vi "485AAA.vi"() -> ()   [LabVIEW 2024]
uses:
  <vilib>/Utility/file.llb/Write Delimited Spreadsheet (string).vi
  <vilib>/Instr/_visa.llb/VISA Configure Serial Port (Instr).vi
panel:
  out "错误输出":errorcluster
  in  "停止":bool
  out "读取缓冲区":string
  out "返回数":u32
  out "波形图表":dbl(graph)
  out "瞬时流量":dbl
  in  "stop bits (10: 1 bit)":u16(ring)=10 caption="停止位（10: 1位）" items=["1.0"=10, "1.5"=15, "2.0"=20]
  in  "parity (0:none)":enum16{"None", "Odd", "Even", "Mark", "Space"}(ring) caption="奇偶（0:无）"
  in  "baud rate (9600)":u32=9600 caption="波特率(9600)"
  in  "VISA resource name":refnum<visa-resource-name> caption="VISA资源名称"
  out "dup path":path caption="路径副本"
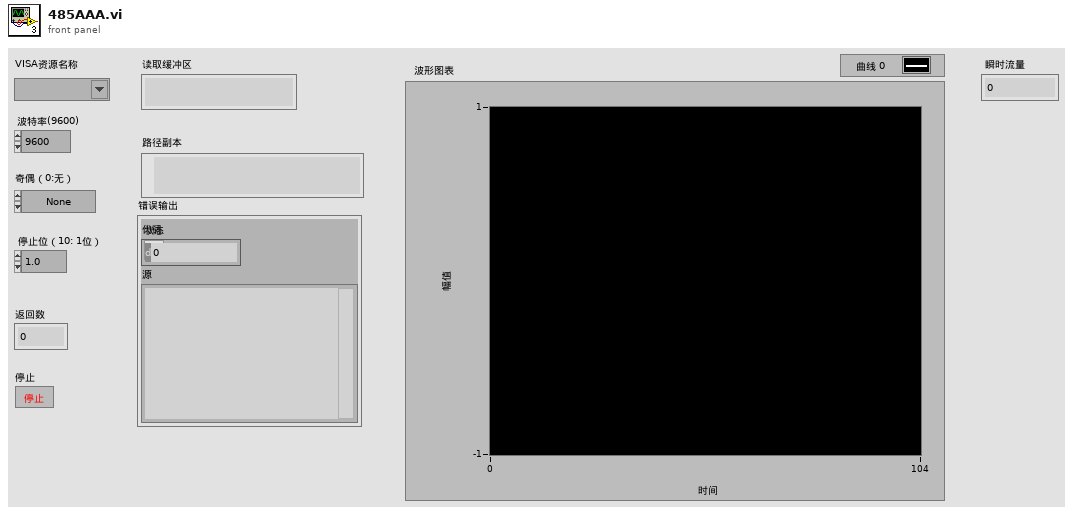
[diagram p1: front panel]
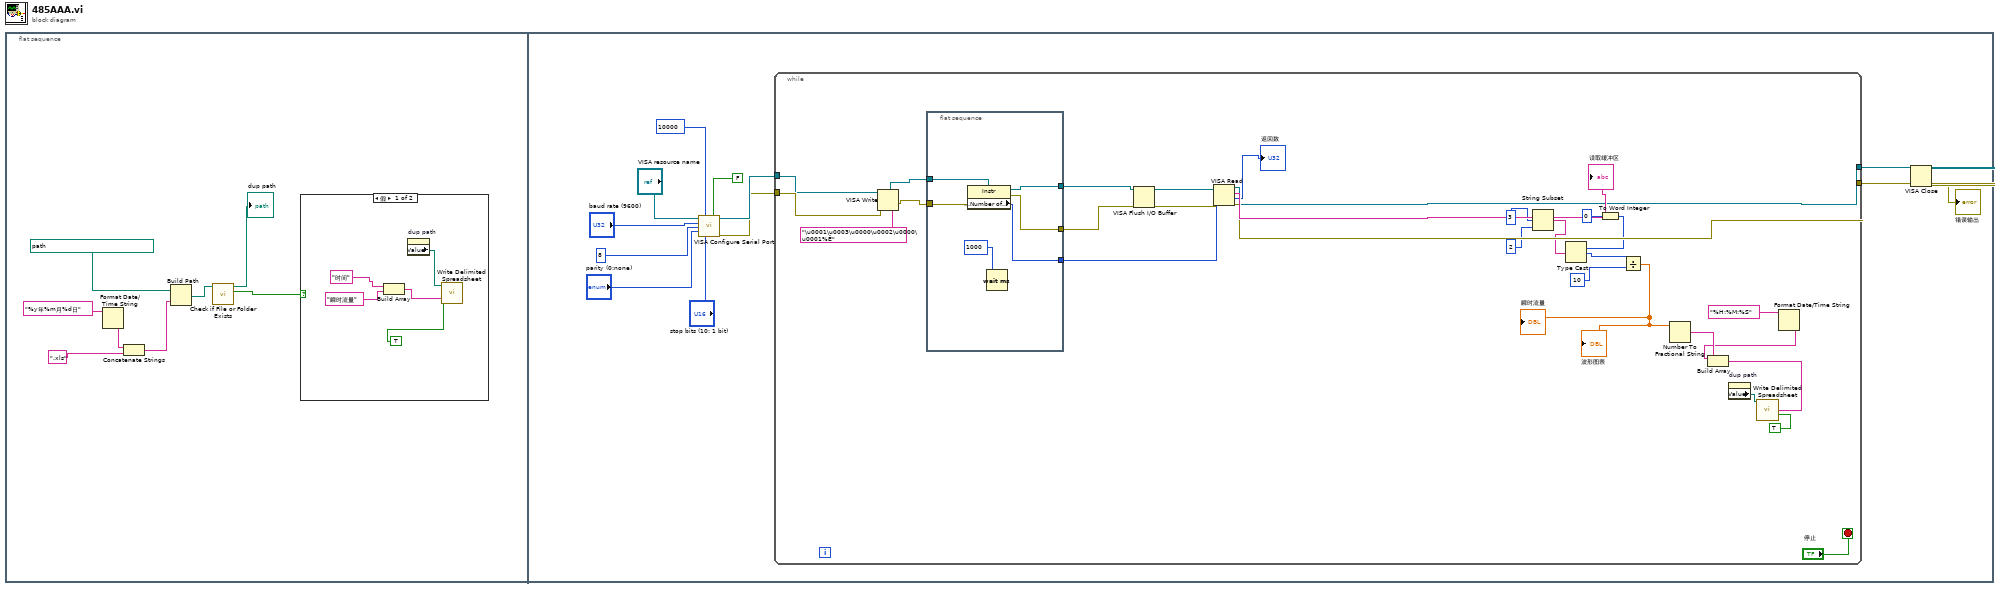
[diagram p0: block diagram]
diagram:
  n1 = flat-sequence {
    frame #0 {
      n2 = Format Date/Time String(time format string (%c)="%y年%m月%d日" ("时间格式字符串(%c)")) -> (date/time string=w6:string)  [unwired: 2 in]
      n3 = Concatenate Strings(w6, ".xls" ("字符串")) -> (w4:string)
      n4 = Build Path(base path=path "C:/Users/AMD/Desktop/数据" ("基路径"), name or relative path=w4) -> (appended path=w3:path)
      n5 = call <vilib>:"Check if File or Folder Exists.vi"("path"=w3) -> ("file or folder exists?"=w1:bool, "dup path"=→"dup path":path)  [unwired: 8 in, 1 out]
      n6 = case shown="假" w1 {
        frame False {
          n7 = Build Array("时间" ("字符串"), "瞬时流量" ("元素")) -> (w11:string[])
          n8 = property on="dup path" class="Path"() -> ("Value"=w9:path)  [unwired: 2 in, 2 out]
          n9 = call-poly <vilib>:"Write Delimited Spreadsheet.vi"("file path (dialog if empty)"=w9, "1D data"=w11, "append to file? (new file:F)"=TRUE) -> ()  [unwired: 11 in, 2 out]
        }
        frame True {
        }
      }
    }
    frame #1 {
      n10 = call-poly "VISA Configure Serial Port"("VISA resource name"="VISA resource name", "timeout (10sec)"=u32 10000, "Enable Termination\nChar (T)"=FALSE ("Enable Termination\nChar (T)"), "baud rate (9600)"="baud rate (9600)", "data bits (8)"=u16 8, "parity (0:none)"="parity (0:none)", "stop bits (10: 1 bit)"="stop bits (10: 1 bit)") -> ("VISA resource name out"=w18:refnum<visa-resource-name>, "error out"=w17:errorcluster)  [unwired: 7 in]
      n11 = while {
        tunnel: w18 -> [w53]
        tunnel: w17 -> [w54]
        tunnel: [w47] -> w16
        tunnel: [w46] -> w15
        stop <- "停止" stop-if-true
        n12 = VISA Write(VISA resource name=w53, write buffer="\u0001\u0003\u0000\u0002\u0000\u0001%Ê" ("写入缓冲区"), error in (no error)=w54) -> (VISA resource name out=w45:refnum<visa-resource-name>, error out=w44:errorcluster)  [unwired: 1 out]
        n13 = flat-sequence {
          tunnel: [w60] -> w52
          tunnel: [w59] -> w51
          tunnel: [w58] -> w50
          tunnel: w45 -> [w57]
          tunnel: w44 -> [w56]
          frame #0 {
            n14 = property class="Instr"(reference=w57, error in=w56) -> (reference out=w60:refnum<visa-resource-name>, error out=w59:errorcluster, "Serial Settings:Number of Bytes at Serial Port"=w58:u32)
            n15 = Wait (ms)(milliseconds to wait=u32 1000 ("等待时间（毫秒）")) -> ()  [unwired: 1 out]
          }
        }
        n16 = VISA Flush I/O Buffer(VISA resource name=w52, error in (no error)=w51) -> (VISA resource name out=w41:refnum<visa-resource-name>, error out=w40:errorcluster)  [unwired: 1 in]
        n17 = VISA Read(VISA resource name=w41, byte count=w50, error in (no error)=w40) -> (VISA resource name out=w47:refnum<visa-resource-name>, read buffer=w49:string, return count=→"返回数":u32, error out=w46:errorcluster)
        "读取缓冲区" <- w49
        n18 = String Subset(string=w49, offset (0)=3 ("偏移量(0)"), length (rest)=2 ("长度（剩余）")) -> (substring=w32:string)
        n19 = To Word Integer(number=i16 0 ("数字")) -> (16bit integer=w33:i16)
        n20 = Type Cast(type=w33, x=w32) -> (*(type *) &x=w34:i16)
        n21 = Divide(x=w34, y=i16 10) -> (x/y=w36:dbl)
        "波形图表" <- w36
        "瞬时流量" <- w36
        n22 = Number To Fractional String(number=w36) -> (F-format string=w39:string)  [unwired: 3 in]
        n23 = property on="dup path" class="Path"() -> ("Value"=w37:path)  [unwired: 2 in, 2 out]
        n24 = Format Date/Time String(time format string (%c)="%H:%M:%S" ("时间格式字符串(%c)")) -> (date/time string=w38:string)  [unwired: 2 in]
        n25 = Build Array(w38, w39) -> (w35:string[])
        n26 = call-poly <vilib>:"Write Delimited Spreadsheet.vi"("file path (dialog if empty)"=w37, "1D data"=w35, "append to file? (new file:F)"=TRUE) -> ()  [unwired: 11 in, 2 out]
      }
      n27 = VISA Close(VISA resource name=w16, error in (no error)=w15) -> (error out=→"错误输出":errorcluster)
    }
  }
